vi "Read_INI_File-Image_Proc.vi"(8 "ERROR IN":errorcluster, 11 "[IN] refnum - ini file":T1) -> (0 "ERROR OUT":errorcluster, 1 "[OUT] Minimal diameter":dbl, 3 "[OUT] Erosion Number":i32, 4 "[OUT] Maximal diameter":dbl, 5 "[OUT] Index for thresholding":i8, 6 "[OUT] Sigma":dbl, 7 "[OUT] Keep Negative Values":bool)   [LabVIEW 2017]
doc: "This subVI reads two values in the *ini file - under the \"Image Processing Values\" section"
uses:
  <vilib>/Utility/config.llb/Config Data RefNum.ctl
  <vilib>/Utility/config.llb/Read Key (I32).vi
  <vilib>/Utility/config.llb/Read Key (Double).vi
  <vilib>/Utility/config.llb/Read Key (Boolean).vi
  <vilib>/Utility/config.llb/NI_LVConfig.lvlib
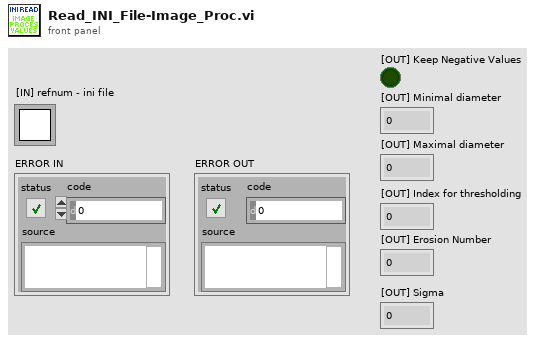
[diagram p1: front panel]
types:
  T1 = typedef "NI_LVConfig.lvlib/Config Data RefNum.ctl" = refnum<k1>
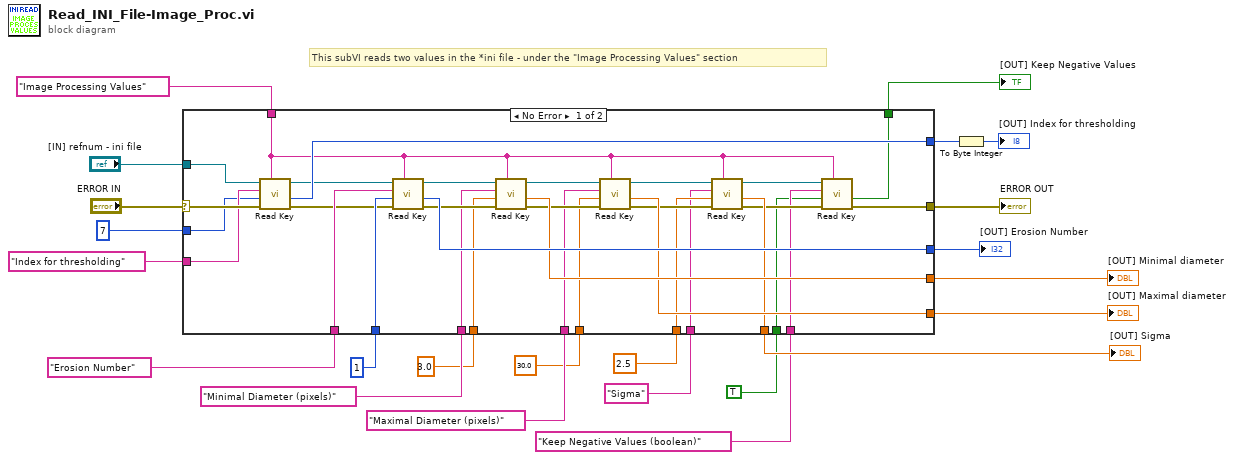
[diagram p0: block diagram]
diagram:
  # "This subVI reads two values in the *ini file - under the \"Image Processing Values\" section"
  n1 = case shown="No Error" "ERROR IN" {
    selector: "ERROR IN" -> [w55 w61]
    tunnel: "[IN] refnum - ini file" -> [w54 _]
    tunnel: "Image Processing Values" ("section") -> [w28 _]
    tunnel: "Index for thresholding" ("key") -> [w53 _]
    tunnel: 7 ("default value") -> [w52 w62]
    tunnel: [w51 w62] -> w15
    tunnel: "Erosion Number" ("key") -> [w49 _]
    tunnel: 1 ("default value") -> [w48 w60]
    tunnel: [w25 w61] -> w16
    tunnel: [w46 w60] -> w13
    tunnel: "Minimal Diameter (pixels)" ("key") -> [w43 _]
    tunnel: 3.0 ("default value") -> [w42 w59]
    tunnel: [w41 w59] -> w10
    tunnel: "Maximal Diameter (pixels)" ("key") -> [w38 _]
    tunnel: 30.0 ("default value") -> [w37 w58]
    tunnel: [w36 w58] -> w7
    tunnel: 2.5 ("default value") -> [w33 w57]
    tunnel: [w32 w57] -> w4
    tunnel: "Sigma" ("key") -> [w31 _]
    tunnel: "Keep Negative Values (boolean)" ("key") -> [w27 _]
    tunnel: TRUE -> [w26 w56]
    tunnel: [w24 w56] -> w1
    frame No Error {
      n2 = call-poly <vilib>:"Read Key.vi"("section"=w28, "error in (no error)"=w55, "default value"=w52, "key"=w53, "refnum"=w54) -> ("error out"=w47:errorcluster, "value"=w51:i32, "refnum out"=w50:T1)  [unwired: 3 in, 1 out]
      n3 = call-poly <vilib>:"Read Key.vi"("section"=w28, "error in (no error)"=w47, "default value"=w48, "key"=w49, "refnum"=w50) -> ("error out"=w44:errorcluster, "value"=w46:i32, "refnum out"=w45:T1)  [unwired: 3 in, 1 out]
      n4 = call-poly <vilib>:"Read Key.vi"("section"=w28, "error in (no error)"=w44, "default value"=w42, "key"=w43, "refnum"=w45) -> ("error out"=w39:errorcluster, "value"=w41:dbl, "refnum out"=w40:T1)  [unwired: 3 in, 1 out]
      n5 = call-poly <vilib>:"Read Key.vi"("section"=w28, "error in (no error)"=w39, "default value"=w37, "key"=w38, "refnum"=w40) -> ("error out"=w34:errorcluster, "value"=w36:dbl, "refnum out"=w35:T1)  [unwired: 3 in, 1 out]
      n6 = call-poly <vilib>:"Read Key.vi"("section"=w28, "error in (no error)"=w34, "default value"=w33, "key"=w31, "refnum"=w35) -> ("error out"=w29:errorcluster, "value"=w32:dbl, "refnum out"=w30:T1)  [unwired: 3 in, 1 out]
      n7 = call-poly <vilib>:"Read Key.vi"("section"=w28, "error in (no error)"=w29, "default value"=w26, "key"=w27, "refnum"=w30) -> ("error out"=w25:errorcluster, "value"=w24:bool)  [unwired: 3 in, 2 out]
    }
    frame Error {
    }
  }
  "ERROR OUT" <- w16
  "[OUT] Erosion Number" <- w13
  "[OUT] Minimal diameter" <- w10
  "[OUT] Maximal diameter" <- w7
  "[OUT] Sigma" <- w4
  "[OUT] Keep Negative Values" <- w1
  n8 = To Byte Integer(number=w15) -> (8bit integer=→"[OUT] Index for thresholding":i8)
